vi "CobotJointTempEquation.vi"(8 "error in (no error)":errorcluster caption="에러 입력(에러 없음)", 11 "CobotJointTempList":i16[](array[numeric])) -> (0 "error out":errorcluster caption="에러 출력", 3 "TempColorArr":u32[](array[numeric]))   [LabVIEW 2019]
uses:
  TempState.ctl
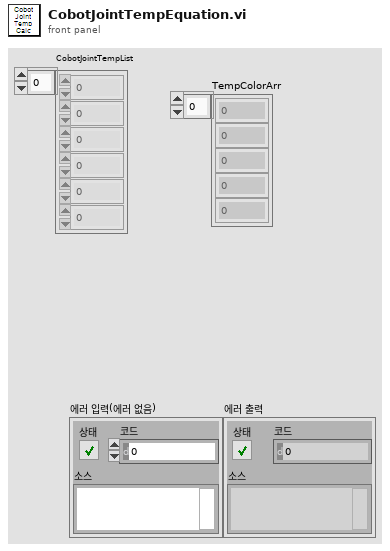
[diagram p1: front panel]
types:
  T1 = typedef "TempState.ctl" = enum16{"정상", "보통", "주의"}
  T2 = cluster{"CobotJointTempList[0]":i16, "CobotJointTempList[1]":i16, "CobotJointTempList[2]":i16, "CobotJointTempList[3]":i16, "CobotJointTempList[4]":i16, "CobotJointTempList[5]":i16, "CobotJointTempList[6]":i16, "CobotJointTempList[7]":i16, "CobotJointTempList[8]":i16}
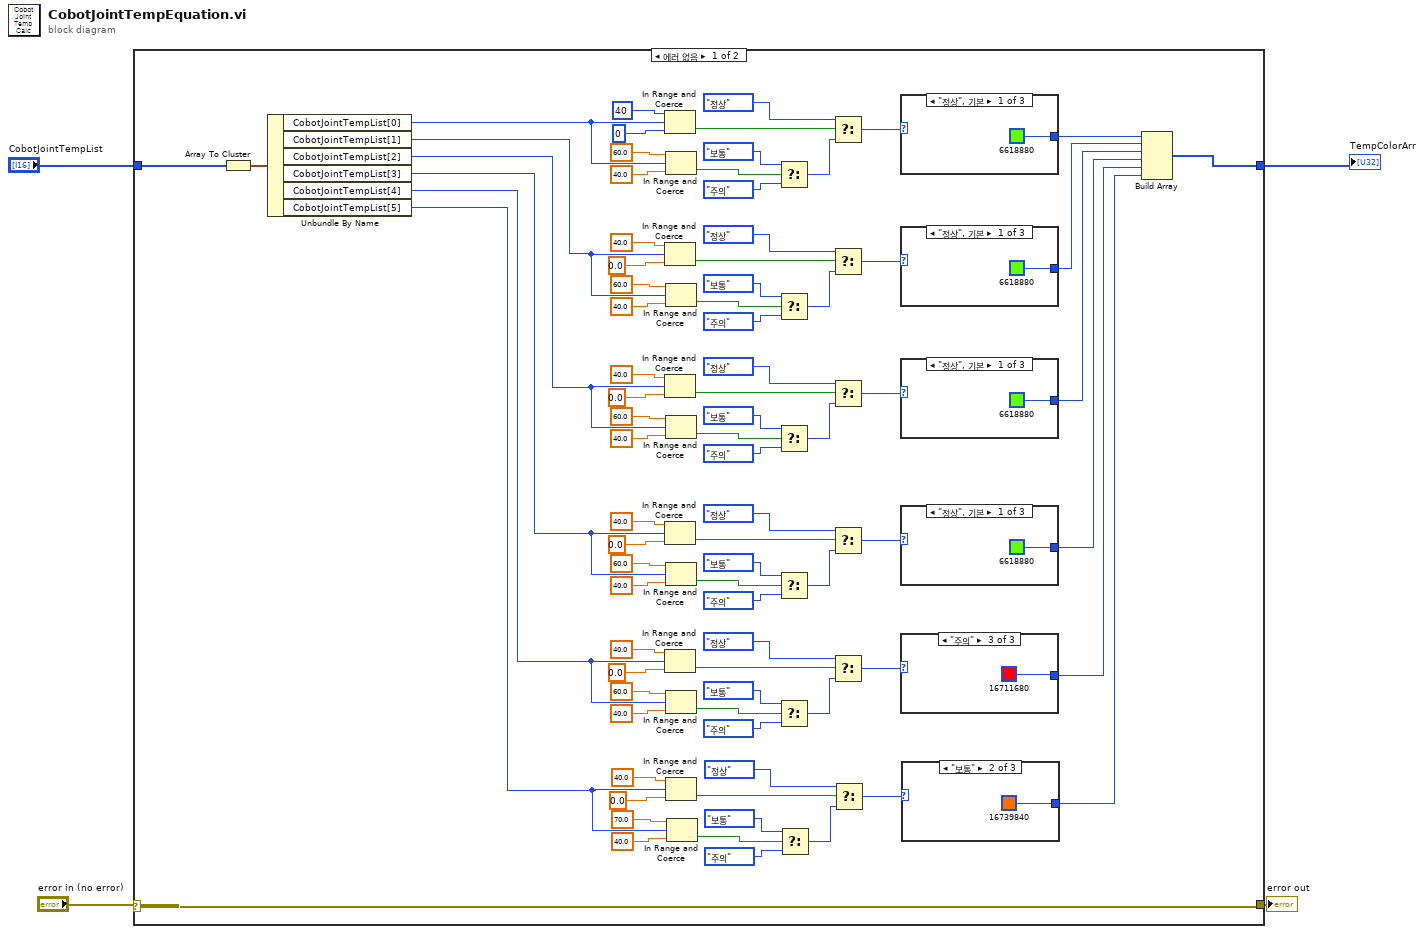
[diagram p0: block diagram]
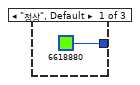
[diagram p2: hidden frame]
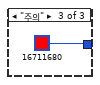
[diagram p3: hidden frame]
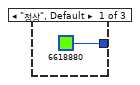
[diagram p4: hidden frame]
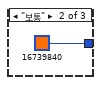
[diagram p5: hidden frame]
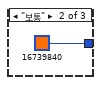
[diagram p6: hidden frame]
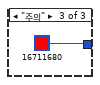
[diagram p7: hidden frame]
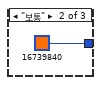
[diagram p8: hidden frame]
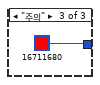
[diagram p9: hidden frame]
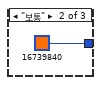
[diagram p10: hidden frame]
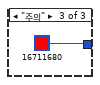
[diagram p11: hidden frame]
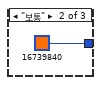
[diagram p12: hidden frame]
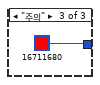
[diagram p13: hidden frame]
diagram:
  n1 = case shown="에러 없음" "error in (no error)" {
    selector: "error in (no error)" -> [w86 w106]
    tunnel: [w86 w106] -> w3
    tunnel: "CobotJointTempList" -> [w6 w105]
    tunnel: [w5 w105] -> w1
    frame No Error {
      n2 = Array To Cluster(array=w6) -> (cluster=w7:T2)
      n3 = Unbundle By Name(w7) -> ("CobotJointTempList[0]"=w74:i16, "CobotJointTempList[1]"=w18:i16, "CobotJointTempList[2]"=w17:i16, "CobotJointTempList[3]"=w16:i16, "CobotJointTempList[4]"=w15:i16, "CobotJointTempList[5]"=w14:i16)
      n4 = In Range and Coerce(upper limit=i16 40 ("상위 리미트"), x=w74, lower limit=i64 0 ("하위 리미트")) -> (In Range?=w75:bool)  [unwired: 1 out]
      n5 = In Range and Coerce(upper limit=40.0 ("상위 리미트"), x=w18, lower limit=0.0 ("하위 리미트")) -> (In Range?=w73:bool)  [unwired: 1 out]
      n6 = In Range and Coerce(upper limit=40.0 ("상위 리미트"), x=w17, lower limit=0.0 ("하위 리미트")) -> (In Range?=w52:bool)  [unwired: 1 out]
      n7 = In Range and Coerce(upper limit=40.0 ("상위 리미트"), x=w16, lower limit=0.0 ("하위 리미트")) -> (In Range?=w51:bool)  [unwired: 1 out]
      n8 = In Range and Coerce(upper limit=40.0 ("상위 리미트"), x=w15, lower limit=0.0 ("하위 리미트")) -> (In Range?=w30:bool)  [unwired: 1 out]
      n9 = In Range and Coerce(upper limit=60.0 ("상위 리미트"), x=w74, lower limit=40.0 ("하위 리미트")) -> (In Range?=w78:bool)  [unwired: 1 out]
      n10 = In Range and Coerce(upper limit=60.0 ("상위 리미트"), x=w18, lower limit=40.0 ("하위 리미트")) -> (In Range?=w70:bool)  [unwired: 1 out]
      n11 = In Range and Coerce(upper limit=60.0 ("상위 리미트"), x=w17, lower limit=40.0 ("하위 리미트")) -> (In Range?=w55:bool)  [unwired: 1 out]
      n12 = In Range and Coerce(upper limit=60.0 ("상위 리미트"), x=w16, lower limit=40.0 ("하위 리미트")) -> (In Range?=w48:bool)  [unwired: 1 out]
      n13 = In Range and Coerce(upper limit=60.0 ("상위 리미트"), x=w15, lower limit=40.0 ("하위 리미트")) -> (In Range?=w33:bool)  [unwired: 1 out]
      n14 = In Range and Coerce(upper limit=40.0 ("상위 리미트"), x=w14, lower limit=0.0 ("하위 리미트")) -> (In Range?=w19:bool)  [unwired: 1 out]
      n15 = In Range and Coerce(upper limit=70.0 ("상위 리미트"), x=w14, lower limit=40.0 ("하위 리미트")) -> (In Range?=w22:bool)  [unwired: 1 out]
      n16 = Select(t=TempState."보통" ("열거형"), s=w78, f=TempState."주의" ("열거형")) -> (s? t:f=w76:T1)
      n17 = Select(t=TempState."보통" ("열거형"), s=w70, f=TempState."주의" ("열거형")) -> (s? t:f=w72:T1)
      n18 = Select(t=TempState."보통" ("열거형"), s=w55, f=TempState."주의" ("열거형")) -> (s? t:f=w53:T1)
      n19 = Select(t=TempState."보통" ("열거형"), s=w48, f=TempState."주의" ("열거형")) -> (s? t:f=w50:T1)
      n20 = Select(t=TempState."보통" ("열거형"), s=w33, f=TempState."주의" ("열거형")) -> (s? t:f=w31:T1)
      n21 = Select(t=TempState."보통" ("열거형"), s=w22, f=TempState."주의" ("열거형")) -> (s? t:f=w20:T1)
      n22 = Select(t=TempState."정상" ("열거형"), s=w75, f=w76) -> (s? t:f=w77:T1)
      n23 = Select(t=TempState."정상" ("열거형"), s=w73, f=w72) -> (s? t:f=w71:T1)
      n24 = Select(t=TempState."정상" ("열거형"), s=w52, f=w53) -> (s? t:f=w54:T1)
      n25 = Select(t=TempState."정상" ("열거형"), s=w51, f=w50) -> (s? t:f=w49:T1)
      n26 = Select(t=TempState."정상" ("열거형"), s=w30, f=w31) -> (s? t:f=w32:T1)
      n27 = Select(t=TempState."정상" ("열거형"), s=w19, f=w20) -> (s? t:f=w21:T1)
      n28 = case shown="\"정상\", 기본" w77 {
        tunnel: [u32 6618880 u32 16739840 u32 16711680] -> w13
        frame "정상", Default {
        }
        frame "보통" {
        }
        frame "주의" {
        }
      }
      n29 = case shown="\"정상\", 기본" w71 {
        tunnel: [u32 6618880 u32 16739840 u32 16711680] -> w12
        frame "정상", Default {
        }
        frame "보통" {
        }
        frame "주의" {
        }
      }
      n30 = case shown="\"정상\", 기본" w54 {
        tunnel: [u32 6618880 u32 16739840 u32 16711680] -> w11
        frame "정상", Default {
        }
        frame "보통" {
        }
        frame "주의" {
        }
      }
      n31 = case shown="\"정상\", 기본" w49 {
        tunnel: [u32 6618880 u32 16739840 u32 16711680] -> w10
        frame "정상", Default {
        }
        frame "보통" {
        }
        frame "주의" {
        }
      }
      n32 = case shown="\"주의\"" w32 {
        tunnel: [u32 6618880 u32 16739840 u32 16711680] -> w9
        frame "정상", Default {
        }
        frame "보통" {
        }
        frame "주의" {
        }
      }
      n33 = case shown="\"보통\"" w21 {
        tunnel: [u32 6618880 u32 16739840 u32 16711680] -> w8
        frame "정상", Default {
        }
        frame "보통" {
        }
        frame "주의" {
        }
      }
      n34 = Build Array(w13, w12, w11, w10, w9, w8) -> (w5:u32[])
    }
    frame Error {
    }
  }
  "error out" <- w3
  "TempColorArr" <- w1
